vi "NanonisDoTTLPulse.vi"(8 "error in (no error)":errorcluster, 11 "String input":string="string test") -> (0 "error out":errorcluster, 3 "String output":string)   [LabVIEW 2011]
uses:
  <userlib>/Nanonis Prog Interface/Nanonis Prog Interface.lvlib
panel:
  in  "Number of pulses (10)":u16=10 max=32767
  in  "Line":dbl[](array[numeric])
  out "Application ref out":refnum<vi>
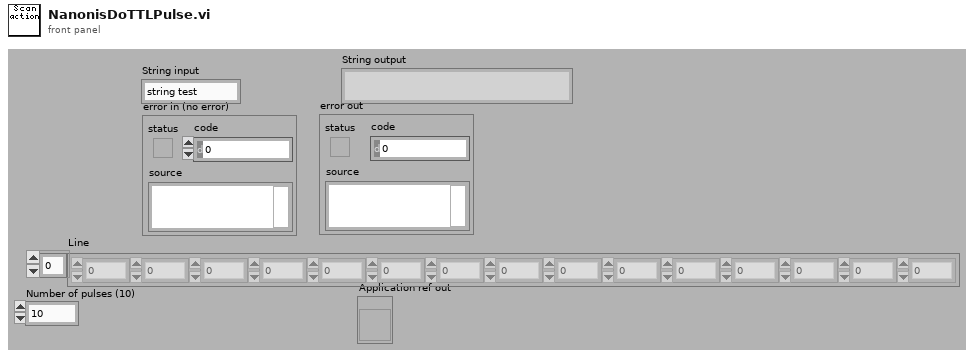
[diagram p1: front panel]
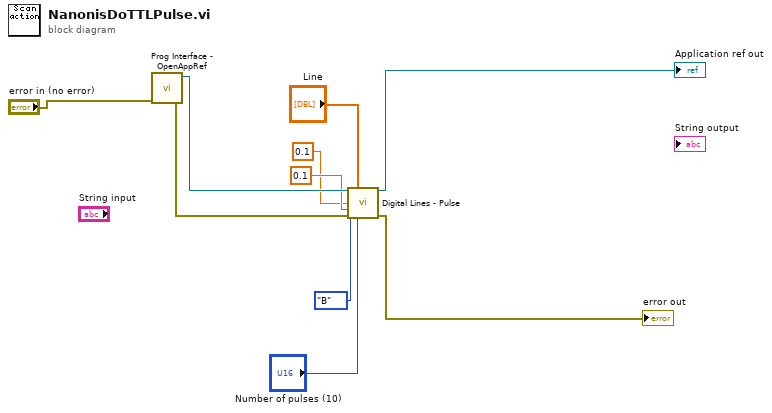
[diagram p0: block diagram]
diagram:
  n1 = call <userlib>:"Prog Interface - OpenAppRef.vi"("Error in (no error)"="error in (no error)") -> ("Error out"=w6:errorcluster, "Application reference"=w9:refnum<vi>)  [unwired: 5 in]
  n2 = call <userlib>:"Digital Lines - Pulse.vi"("Application ref in"=w9, "Digital lines (1-8)"="Line", "Port (A)"=enum16{"A", "B"}."B", "Pulse width (s)"=0.1, "Pulse pause (s)"=0.1, "Error in (no error)"=w6, "Number of pulses (10)"="Number of pulses (10)") -> ("Application ref out"=→"Application ref out":refnum<vi>, "Error out"=→"error out":errorcluster)  [unwired: 6 in, 1 out]
